vi "to string.vi"(8 "error in":errorcluster, 11 "fixed channel configuration in":refnum<class "control module configuration.lvclass">=refnum) -> (0 "error out":errorcluster, 1 "data":string, 2 "version":string, 3 "fixed channel configuration out":refnum<class "control module configuration.lvclass">)   [LabVIEW 2014, in "control module configuration.lvclass"]
doc: "Provides an interface for saving a module configuration to a file or other serialized data source. It is recommended that all children of this class store data in two sets--data required for its own initialization, and any data required for parent initialization--and that each implementation uses the <b>Call Parent Method</b> primitive to serialize parent information.\nNI Tag Bus Module Framework 1.0.3.43\nNI Systems Engineering"
uses:
  control module configuration.lvclass
  <vilib>/NI/Tag Bus Module Framework/channel/TBM channel.lvclass
  <vilib>/NI/Configuration Framework/serializable configuration/NISE_CEF_serializable configuration.lvclass
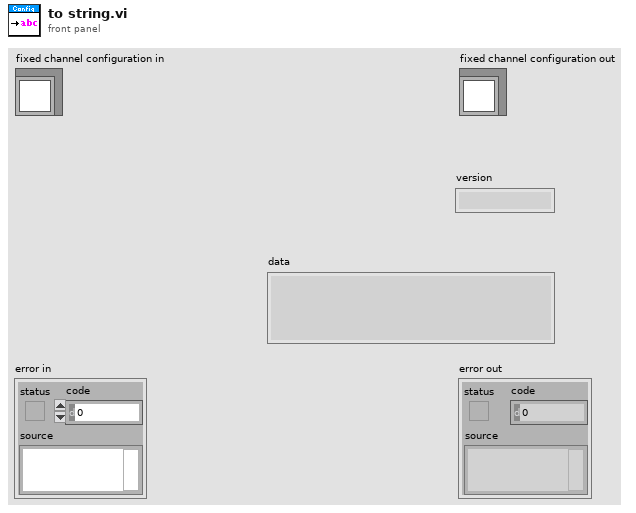
[diagram p1: front panel]
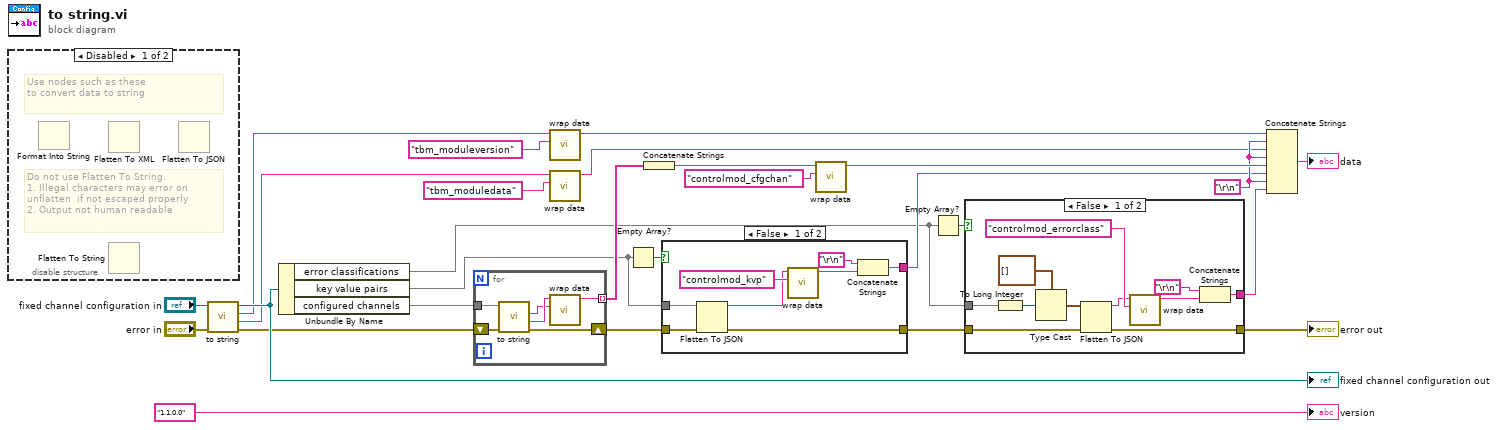
[diagram p0: block diagram]
diagram:
  w6 = "\r\n"
  n1 = disable-structure shown="Disabled" {
    frame Disabled {
      # "Do not use Flatten To String.\n1. Illegal characters may error on unflatten  if not escaped properly\n2. Output not human readable"
      # "Use nodes such as these \nto convert data to string"
      n2 = Format Into String() -> ()  [unwired: 4 in, 2 out]
      n3 = Flatten To XML() -> ()  [unwired: 1 in, 1 out]
      n4 = Flatten To String() -> ()  [unwired: 4 in, 3 out]
      n5 = Flatten To JSON() -> ()  [unwired: 3 in, 2 out]
    }
    frame Enabled {
    }
  }
  n6 = call-parent "to string.vi"("error in"="error in", "module configuration in"="fixed channel configuration in") -> ("error out"=w23:errorcluster, "data"=w16:string, "version"=w15:string, "module configuration out"=w25:refnum<class "control module configuration.lvclass">)  [unwired: 6 in]
  "fixed channel configuration out" <- w25
  n7 = Unbundle By Name(w25) -> ("error classifications"=w1, "key value pairs"=w11, "configured channels"=w2)
  n8 = for {
    tunnel: w2 -> [w33]
    shift-right: [w29] -> w10
    shift-left: w23 -> [w30]
    tunnel: [w28] -> w19 mode=indexing
    n9 = call-dynamic "to string.vi"("error in"=w30, "channel in"=w33) -> ("error out"=w29:errorcluster, "channel data"=w32:string, "identifier"=w31:string)  [unwired: 6 in, 1 out]
    n10 = call <vilib>:"wrap data.vi"("identifier"=w31, "data to wrap"=w32) -> ("wrapped data"=w28:string)  [unwired: 9 in]
  }
  n11 = call <vilib>:"wrap data.vi"("identifier"="tbm_moduleversion", "data to wrap"=w15) -> ("wrapped data"=w17:string)  [unwired: 9 in]
  n12 = call <vilib>:"wrap data.vi"("identifier"="tbm_moduledata", "data to wrap"=w16) -> ("wrapped data"=w3:string)  [unwired: 9 in]
  n13 = Empty Array?(array=w11) -> (empty?=w12:bool)
  n14 = Concatenate Strings(w19) -> (w18:string)
  n15 = case shown="False" w12 {
    tunnel: [w39 _] -> w4
    tunnel: w11 -> [w36 _]
    tunnel: w10 -> [w37 w42]
    tunnel: [w34 w42] -> w9
    frame False {
      n16 = Flatten To JSON(anything=w36, error in (no error)=w37) -> (JSON string=w35:string, 11:w34:errorcluster)  [unwired: 1 in]
      n17 = call <vilib>:"wrap data.vi"("identifier"="controlmod_kvp", "data to wrap"=w35) -> ("wrapped data"=w40:string)  [unwired: 9 in]
      n18 = Concatenate Strings("\r\n", w40) -> (w39:string)
    }
    frame True {
    }
  }
  n19 = call <vilib>:"wrap data.vi"("identifier"="controlmod_cfgchan", "data to wrap"=w18) -> ("wrapped data"=w22:string)  [unwired: 9 in]
  n20 = Empty Array?(array=w1) -> (empty?=w5:bool)
  n21 = case shown="False" w5 {
    tunnel: [w51 _] -> w7
    tunnel: w9 -> [w50 w54]
    tunnel: [w48 w54] -> w8
    tunnel: w1 -> [w45 _]
    frame False {
      n22 = To Long Integer(number=w45) -> (32bit integer=w47:i32)
      n23 = Type Cast(type=cluster{i32, i32}[] [], x=w47) -> (*(type *) &x=w44:cluster{i32, i32}[])
      n24 = Flatten To JSON(anything=w44, error in (no error)=w50) -> (JSON string=w49:string, 11:w48:errorcluster)  [unwired: 1 in]
      n25 = call <vilib>:"wrap data.vi"("identifier"="controlmod_errorclass", "data to wrap"=w49) -> ("wrapped data"=w52:string)  [unwired: 9 in]
      n26 = Concatenate Strings("\r\n", w52) -> (w51:string)
    }
    frame True {
    }
  }
  "error out" <- w8
  n27 = Concatenate Strings(w17, w6, w3, w6, w22, w4, w6, w7) -> (→"data":string)
  "version" <- "1.1.0.0" ("version")
